vi "Read polarimeitrc status.vi"(8 "error in (no error)":errorcluster, 11 "S4ICS in":refnum<class "S4ICS.lvclass">) -> (0 "error out":errorcluster, 2 "polarimeitrc status":T1={"waveplate positions"={"WP 1"=TRUE, "WP 2"=FALSE, "WP 3"=FALSE, "WP 4"=FALSE, "WP 5"=FALSE, "WP 6"=FALSE, "WP 9"=FALSE, "WP 8"=FALSE, "WP 7"=FALSE, "WP 10"=FALSE, "WP 11"=FALSE, "WP 12"=FALSE, "WP 13"=FALSE, "WP 14"=FALSE, "WP 15"=FALSE, "WP 16"=FALSE}, "waveplate"=0, "calib wheel"=0} {"calib wheel" items=["OFF", "POLARIZER", "PINHOLE", "SHUTTER", "DEPOLARIZER"]; "waveplate" items=["OFF", "L2", "L4"]}, 3 "S4ICS out":refnum<class "S4ICS.lvclass">)   [LabVIEW 2018, in "S4ICS.lvclass"]
uses:
  S4ICS.lvclass
  S4ICS.lvclass/S4ICS.ctl
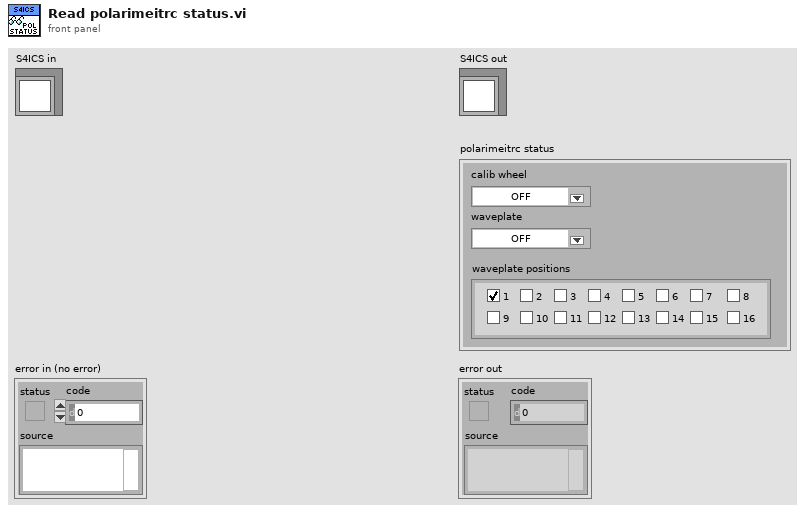
[diagram p1: front panel]
types:
  T1 = cluster{"waveplate positions":cluster{"WP 1":bool, "WP 2":bool, "WP 3":bool, "WP 4":bool, "WP 5":bool, "WP 6":bool, "WP 9":bool, "WP 8":bool, "WP 7":bool, "WP 10":bool, "WP 11":bool, "WP 12":bool, "WP 13":bool, "WP 14":bool, "WP 15":bool, "WP 16":bool}, "waveplate":u16, "calib wheel":u16}
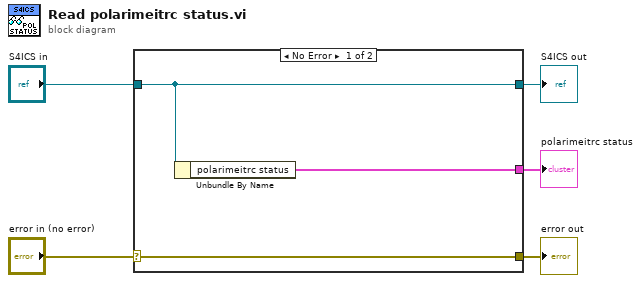
[diagram p0: block diagram]
diagram:
  n1 = case shown="No Error" "error in (no error)" {
    selector: "error in (no error)" -> [w8 w9]
    tunnel: [w8 w9] -> w4
    tunnel: [w7 w10] -> w2
    tunnel: "S4ICS in" -> [w7 w10]
    tunnel: [w6 _] -> w1
    frame No Error {
      n2 = Unbundle By Name(w7) -> ("polarimeitrc status"=w6:T1)
    }
    frame Error {
    }
  }
  "error out" <- w4
  "S4ICS out" <- w2
  "polarimeitrc status" <- w1
